vi "Create.vi"(8 "error in (no error)":errorcluster, 10 "Name":string, 11 "object in":refnum<class "Channel.lvclass">) -> (0 "error out":errorcluster, 3 "object out":refnum<class "Channel.lvclass">)   [LabVIEW 2021, in "Channel.lvlib" / "Channel.lvclass"]
doc: "Creates the Channel"
uses:
  Channel.lvclass
  Channel.lvclass/Channel.ctl
  Configuration_class/Configuration.lvclass
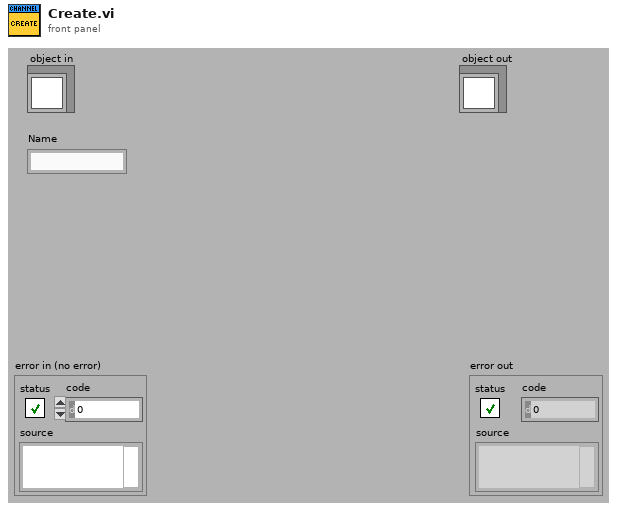
[diagram p1: front panel]
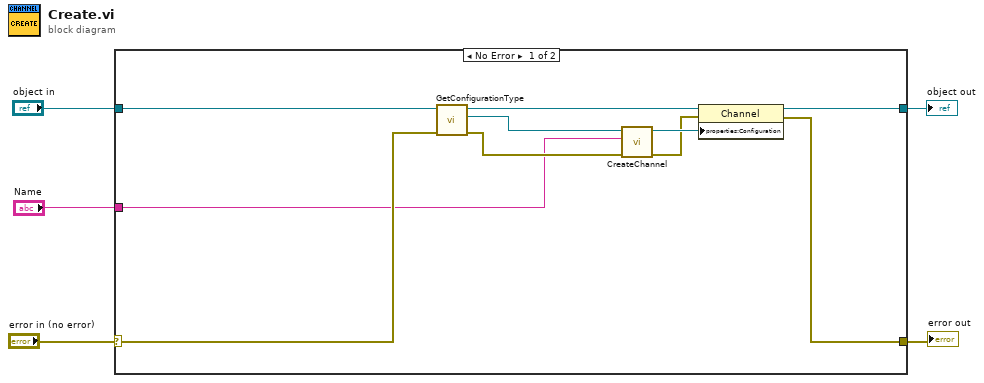
[diagram p0: block diagram]
diagram:
  n1 = case shown="No Error" "error in (no error)" {
    selector: "error in (no error)" -> [w13 w17]
    tunnel: [w7 w17] -> w4
    tunnel: [w12 w16] -> w2
    tunnel: "object in" -> [w15 w16]
    tunnel: "Name" -> [w6 _]
    frame No Error {
      n2 = call-dynamic "GetConfigurationType.vi"("error in (no error)"=w13, "object in"=w15) -> ("error out"=w9:errorcluster, "Configuration"=w11:refnum<class "Configuration.lvclass">, "object out"=w14:refnum<class "Channel.lvclass">)  [unwired: 7 in]
      n3 = call "CreateChannel.vi"("error in (no error)"=w9, "Name"=w6, "object in"=w11) -> ("error out"=w8:errorcluster, "object out"=w10:refnum<class "Configuration.lvclass">)  [unwired: 7 in]
      n4 = property class="Channel"(reference=w14, error in=w8, "properties:Configuration"=w10) -> (reference out=w12:refnum<class "Channel.lvclass">, error out=w7:errorcluster)
    }
    frame Error {
    }
  }
  "error out" <- w4
  "object out" <- w2
